vi "Data Read.vi"(6 "Append Index":i32 min=-1, 8 "error in (no error)":errorcluster, 11 "path":path) -> (0 "error out":errorcluster, 1 "Notes":string, 2 "Data (Dictionary)":T1[](array[typedef]), 3 "path out":path)   [LabVIEW 2019, in "LV-Data.lvclass"]
uses:
  LV-Data.lvclass
  Typedefs/Dictionary--cluster.ctl
  Typedefs/Operation--enum.ctl
  Typedefs/File Type--enum.ctl
panel:
  out "x-y":dbl
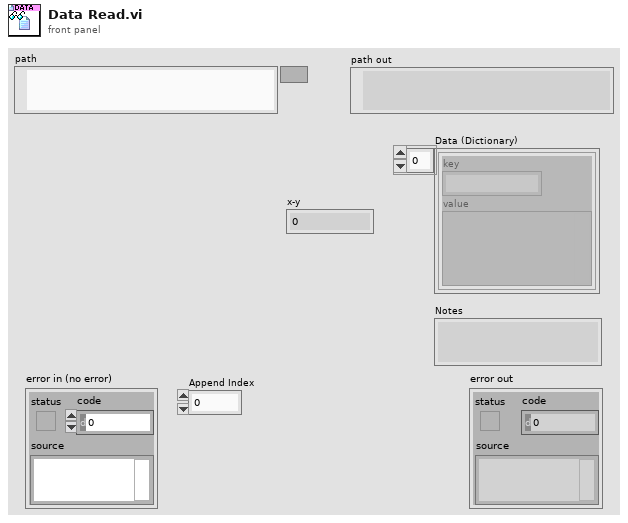
[diagram p1: front panel]
types:
  T1 = typedef "LV-Data.lvclass/Dictionary--cluster.ctl" = cluster{"key":string, "value":variant}
  T2 = typedef "LV-Data.lvclass/Operation--enum.ctl" = enum16{"Read", "Write", "Write + Append"}
  T3 = typedef "LV-Data.lvclass/File Type--enum.ctl" = enum16{"DAT", "ITX", "TDMS", "VI"}
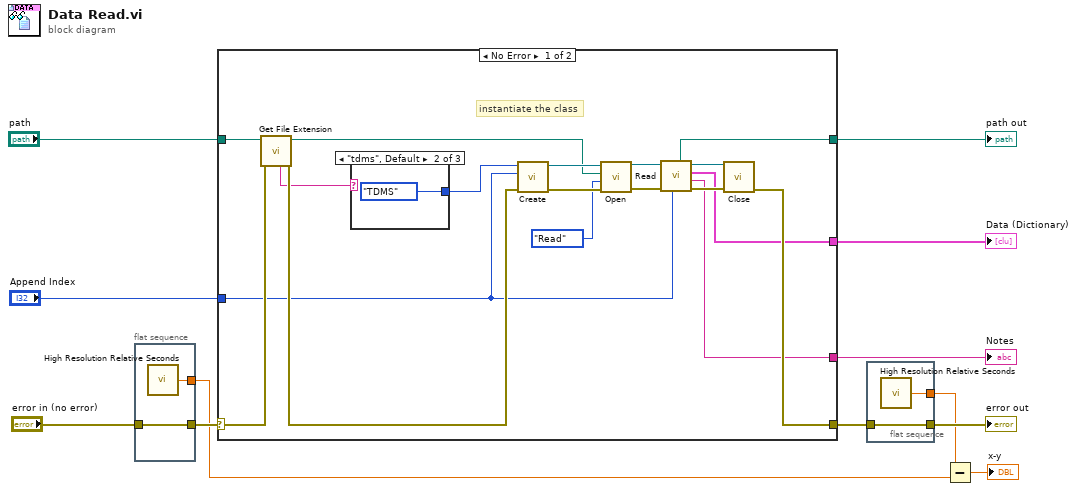
[diagram p0: block diagram]
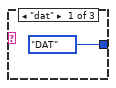
[diagram p2: hidden frame]
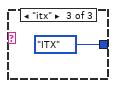
[diagram p3: hidden frame]
diagram:
  n1 = flat-sequence {
    tunnel: "error in (no error)" -> [w14]
    tunnel: [w14] -> w4
    tunnel: [w13] -> w2
    frame #0 {
      n2 = call <vilib>:"High Resolution Relative Seconds.vi"() -> ("relative seconds"=w13:dbl)
    }
  }
  n3 = case shown="No Error" w4 {
    selector: w4 -> [w22 w37]
    tunnel: [w26 w37] -> w7
    tunnel: [w25 w36] -> w12
    tunnel: "path" -> [w20 w36]
    tunnel: [w24 _] -> w9
    tunnel: [w23 _] -> w10
    tunnel: "Append Index" -> [w17 _]
    frame No Error {
      # "instantiate the class"
      n4 = call <vilib>:"Get File Extension.vi"("error in (no error)"=w22, "file"=w20) -> ("error out"=w21:errorcluster, "dup file"=w16:path, "unmodified file extension"=w19:string)  [unwired: 5 in, 2 out]
      n5 = case shown="\"tdms\", Default" w19 {
        tunnel: [File_Type--enum."DAT" ("File Type") File_Type--enum."TDMS" ("File Type") File_Type--enum."ITX" ("File Type")] -> w18
        frame "dat" {
        }
        frame "tdms", Default {
        }
        frame "itx" {
        }
      }
      n6 = call "Create.vi"("error in (no error)"=w21, "Append Index (-1)"=w17, "File Type"=w18) -> ("error out"=w31:errorcluster, "Data out"=w32:refnum<class "LV-Data.lvclass">)  [unwired: 7 in]
      n7 = call-dynamic "Open.vi"("error in (no error)"=w31, "Operation"=Operation--enum."Read", "Path"=w16, "Data in"=w32) -> ("error out"=w29:errorcluster, "Data out"=w30:refnum<class "LV-Data.lvclass">)  [unwired: 6 in]
      n8 = call-dynamic "Read.vi"("Append Index"=w17, "error in (no error)"=w29, "Data Save in"=w30) -> ("error out"=w28:errorcluster, "Notes"=w23:string, "Data (Dictionary)"=w24:T1[], "Data Save out"=w27:refnum<class "LV-Data.lvclass">, "Path out"=w25:path)  [unwired: 4 in]
      n9 = call-dynamic "Close.vi"("error in (no error)"=w28, "Data in"=w27) -> ("error out"=w26:errorcluster)  [unwired: 8 in, 1 out]
    }
    frame Error {
    }
  }
  "path out" <- w12
  "Data (Dictionary)" <- w9
  "Notes" <- w10
  n10 = flat-sequence {
    tunnel: w7 -> [w39]
    tunnel: [w39] -> w6
    tunnel: [w38] -> w3
    frame #0 {
      n11 = call <vilib>:"High Resolution Relative Seconds.vi"() -> ("relative seconds"=w38:dbl)
    }
  }
  n12 = Subtract(x=w3, y=w2) -> (x-y=→"x-y":dbl)
  "error out" <- w6
